vi "Exo_moyenne_boucle.vi"(4 "Entree_tableau":dbl) -> (10 "mean":dbl format="%0.2f")   [LabVIEW 2012]
uses:
  <vilib>/Analysis/baseanly.llb/Mean (DBL).vi
  <vilib>/Analysis/NI_AALBase.lvlib
panel:
  out "x+y":dbl
  out "Array":dbl[](array[numeric])
  out "Numeric":i32
  in  "stop":bool
  out "Waveform Chart":dbl(graph)
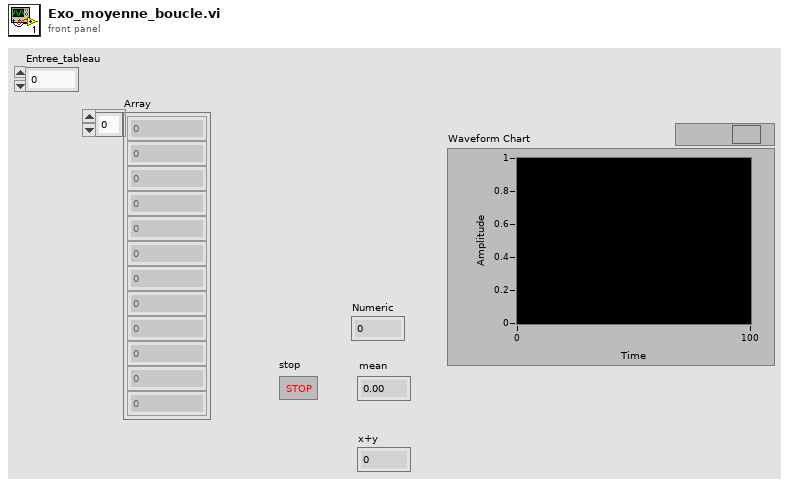
[diagram p1: front panel]
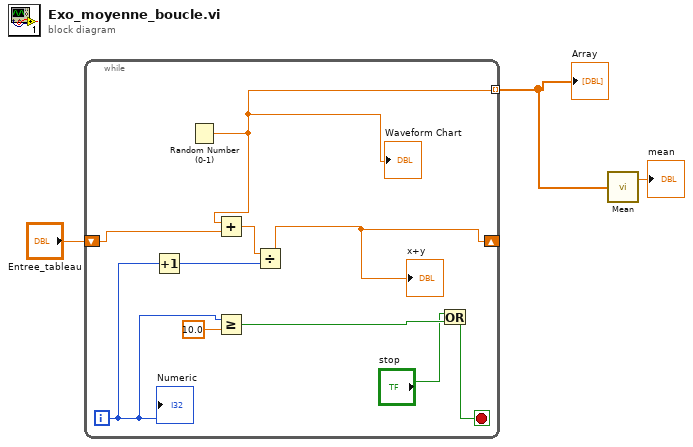
[diagram p0: block diagram]
diagram:
  n1 = while {
    shift-right: [w7] -> _
    shift-left: "Entree_tableau" -> [w9]
    tunnel: [w8] -> w2 mode=indexing
    i -> [w5]
    stop <- w10 stop-if-true
    n2 = Increment(x=w5) -> (x+1=w4:i32)
    n3 = Random Number (0-1)() -> (number: 0 to 1=w8:dbl)
    "Waveform Chart" <- w8
    n4 = Add(x=w8, y=w9) -> (x+y=w6:dbl)
    n5 = Greater Or Equal?(x=w5, y=10.0) -> (x >= y?=w12:bool)
    n6 = Divide(x=w6, y=w4) -> (x/y=w7:dbl)
    "x+y" <- w7
    n7 = Or(x="stop", y=w12) -> (x .or. y?=w10:bool)
    "Numeric" <- w5
  }
  "Array" <- w2
  n8 = call-poly <vilib>:"Mean.vi"("X"=w2) -> ("mean"=→"mean":dbl)  [unwired: 1 out]
